vi "Main_Dashboard.vi"() -> ()   [LabVIEW 2026]
uses:
  <vilib>/Utility/file.llb/Read Delimited Spreadsheet (DBL).vi
  <vilib>/ptbypt/NI_PtbyPt.lvlib
panel:
  out "Detection History Log":string[][](table)
  out "Acitve Node  B":dbl
  out "Acitve Node A":dbl
  in  "CSV File Path":path
  in  "stop":bool
  out "Network Topology Map":cluster{dbl[], dbl[]}[](graph)
  out "Detection Status":string
  out "Wormhole Attack Alarm":bool
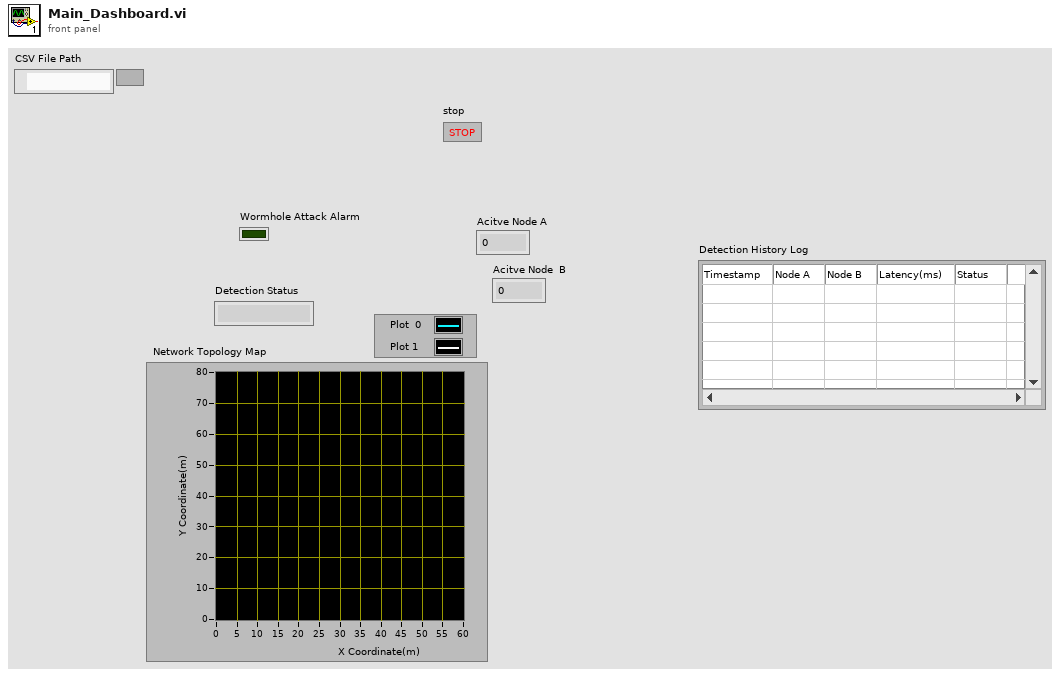
[diagram p1: front panel]
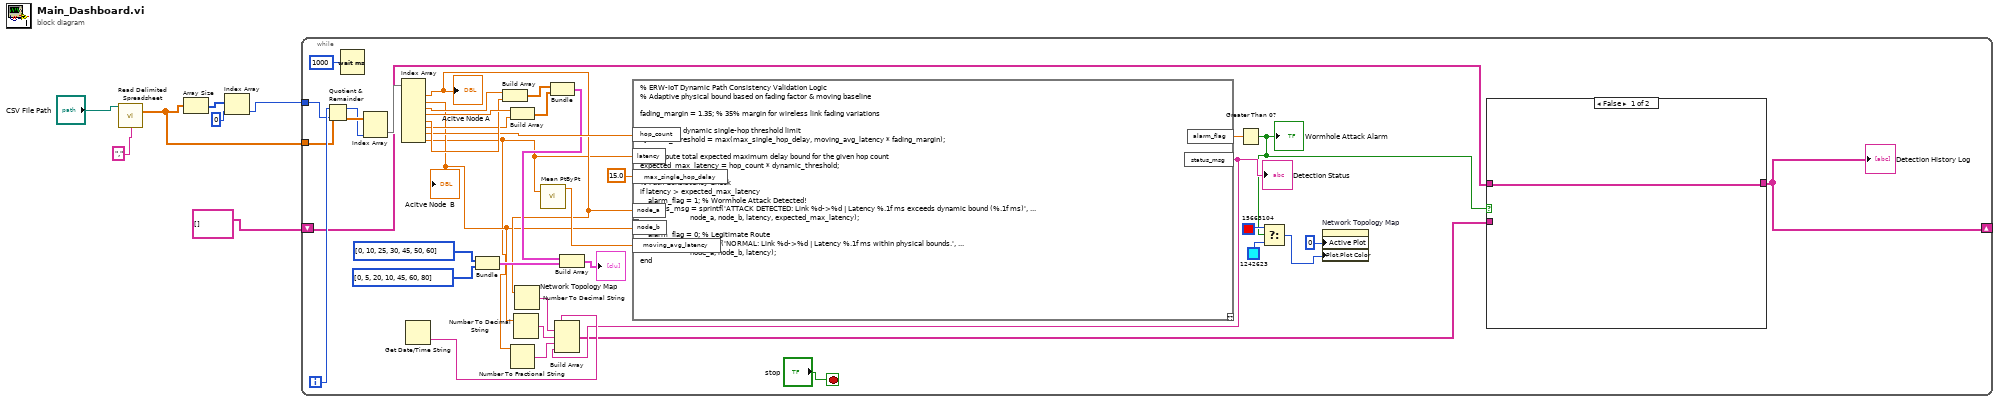
[diagram p0: block diagram]
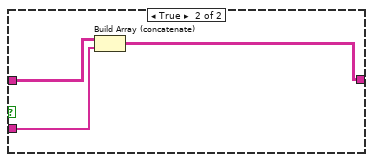
[diagram p2: hidden frame]
diagram:
  n1 = call-poly <vilib>:"Read Delimited Spreadsheet.vi"("file path (dialog if empty)"="CSV File Path", "delimiter (\\t)"="," ("delimiter (\\t)")) -> ("all rows"=w2:dbl[][])  [unwired: 8 in, 5 out]
  n2 = Array Size(array=w2) -> (size(s)=w5:i32[])
  n3 = Index Array(array=w5, index=0) -> (element=w3:i32)
  n4 = while {
    tunnel: w3 -> [w33]
    tunnel: w2 -> [w32]
    shift-right: [w8] -> _
    shift-left: string[][] [] -> [w10]
    i -> [w34]
    stop <- "stop" stop-if-true
    n5 = Quotient & Remainder(x=w34, y=w33) -> (x-y*floor(x/y)=w31:i32)  [unwired: 1 out]
    n6 = Wait (ms)(milliseconds to wait=u32 1000) -> ()  [unwired: 1 out]
    n7 = Index Array(array=w32, index (col)=w31) -> (element=w30:dbl[])  [unwired: 1 in]
    n8 = Index Array(array=w30) -> (element #1=w19:dbl, element #2=w18:dbl, element #3=w40:dbl, element #4=w39:dbl, element #5=w38:dbl, element #6=w37:dbl, element #7=w36:dbl, element #8=w17:dbl)  [unwired: 8 in]
    "Acitve Node A" <- w19
    "Acitve Node  B" <- w18
    n9 = Get Date/Time String() -> (time string=w16:string)  [unwired: 3 in, 1 out]
    n10 = Bundle(i32[] [0, 10, 25, 30, 45, 50, 60], i32[] [0, 5, 20, 10, 45, 60, 80]) -> (w24:cluster{i32[], i32[]})  [unwired: 1 in]
    n11 = Build Array(w40, w38) -> (w42:dbl[])
    n12 = Build Array(w39, w37) -> (w41:dbl[])
    n13 = Number To Fractional String(number=w17) -> (F-format string=w13:string)  [unwired: 3 in]
    n14 = Number To Decimal String(number=w18) -> (decimal integer string=w14:string)  [unwired: 1 in]
    n15 = Number To Decimal String(number=w19) -> (decimal integer string=w15:string)  [unwired: 1 in]
    n16 = call <vilib>:"Mean PtByPt.vi"("x"=w17) -> ("mean"=w29:dbl)  [unwired: 3 in, 1 out]
    n17 = Bundle(w42, w41) -> (w26:cluster{dbl[], dbl[]})  [unwired: 1 in]
    n18 = Build Array(w26, w24) -> (→"Network Topology Map":cluster{dbl[], dbl[]}[])
    n19 = script code="% ERW-IoT Dynamic Path Consistency Validation Logic\n% Adaptive physical bound based on fading factor & moving baseline\n\nfading_margin = 1.35; % 35% margin for wireless link fading variations\n\n% Calculate dynamic single-hop threshold limit\ndynamic_threshold = max(max_single_hop_delay, moving_avg_latency * fading_margin);\n\n% Compute total expected maximum delay bound for the given hop count\nexpected_max_latency = hop_count * dynamic_threshold;\n\n% Path Consistency Check\nif latency > expected_max_latency\n    alarm_flag = 1; % Wormhole Attack Detected!\n    status_msg = sprintf('ATTACK DETECTED: Link %d->%d | Latency %.1f ms exceeds dynamic bound (%.1f ms)', ...\n                         node_a, node_b, latency, expected_max_latency);\nelse\n    alarm_flag = 0; % Legitimate Route\n    status_msg = sprintf('NORMAL: Link %d->%d | Latency %.1f ms within physical bounds.', ...\n                         node_a, node_b, latency);\nend"("hop_count"=w36, "latency"=w17, "max_single_hop_delay"=15.0 ("Real"), "node_a"=w19, "node_b"=w18, "moving_avg_latency"=w29) -> ("alarm_flag"=w43:dbl, "status_msg"=w12:string)  [unwired: 1 in, 1 out]
    "Detection Status" <- w12
    n20 = Build Array(w16, w15, w14, w13, w12) -> (w9:string[])
    n21 = Greater Than 0?(x=w43) -> (x > 0?=w11:bool)
    "Wormhole Attack Alarm" <- w11
    n22 = Select(t=u32 15663104, s=w11, f=u32 1242623) -> (s? t:f=w20:u32)
    n23 = property on="Network Topology Map" class="XYGraph (strict)"("Active Plot"=u32 0, "Plot.Plot Color"=w20) -> ()  [unwired: 2 in, 2 out]
    n24 = case shown="False" w11 {
      tunnel: w10 -> [w46 w49]
      tunnel: w9 -> [_ w48]
      tunnel: [w46 w47] -> w8
      frame False {
      }
      frame True {
        n25 = Build Array (concatenate)(w49, w48) -> (w47:string[][])
      }
    }
    "Detection History Log" <- w8
  }
